vi "Configure Session.vi"(8 "error in":errorcluster, 11 "Plugin in":refnum<class "DateTimeChannel.lvclass">) -> (0 "error out":errorcluster, 3 "Plugin out":refnum<class "DateTimeChannel.lvclass">)   [LabVIEW 2023, in "DateTimeChannel.lvlib" / "DateTimeChannel.lvclass"]
uses:
  DateTimeChannel.lvclass
  C:/Program Files/National Instruments/LabVIEW 2023/vi.lib/FlexLogger/SDK/PluginSDK.lvlibp/PEFClasses/SDK/Plugin/Plugin.lvclass
  DateTimeChannel.lvclass/DateTimeChannel.ctl
  Date Time Channel Global.vi
  <vilib>/FlexLogger/SDK/PluginSDK.lvlibp/PEFClasses/SDK/Plugin/ParameterAccess/Read String.vi
  <vilib>/FlexLogger/SDK/PluginSDK.lvlibp/PEFClasses/SDK/Plugin/Plugin.lvclass
  C:/Program Files/National Instruments/LabVIEW 2023/vi.lib/FlexLogger/SDK/PluginSDK.lvlibp/PEFClasses/SDK/Processing Element/Processing Element.lvclass
  C:/dev/niflexlogger-plugins/plugins/DateTimeChannel/source/DateTimeChannel/DateTimeChannel.lvclass
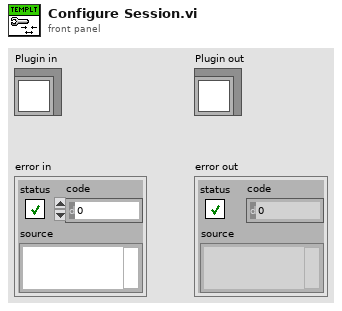
[diagram p1: front panel]
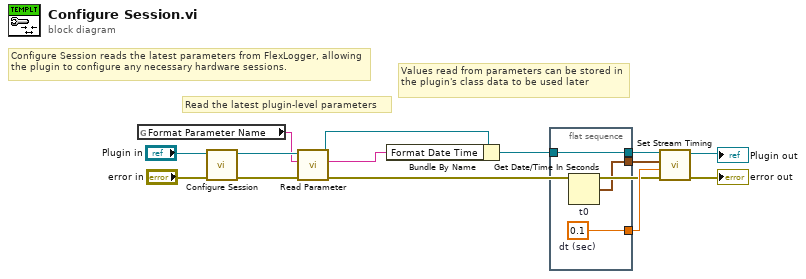
[diagram p0: block diagram]
diagram:
  # "Read the latest plugin-level parameters"
  # "Configure Session reads the latest parameters from FlexLogger, allowing the plugin to configure any necessary hardware sessions."
  # "Values read from parameters can be stored in the plugin's class data to be used later"
  n1 = global read "Date Time Channel Global.vi" "Format Parameter Name"() -> (w1:string)
  n2 = call-parent "Configure Session.vi"("error in (no error)"="error in", "Processing Element in"="Plugin in") -> ("error out"=w7:errorcluster, "Processing Element out"=w8:refnum<class "DateTimeChannel.lvclass">)  [unwired: 8 in]
  n3 = call-poly <vilib>:"Read Parameter.vi"("error in (no error)"=w7, "Name"=w1, "Plugin in"=w8) -> ("error out"=w4:errorcluster, "Value"=w5:string, "Plugin out"=w6:refnum<class "DateTimeChannel.lvclass">)  [unwired: 5 in, 1 out]
  n4 = Bundle By Name(cluster=w6, "Format Date Time"=w5) -> (w11:refnum<class "DateTimeChannel.lvclass">)
  n5 = flat-sequence {
    tunnel: [w17] -> w10
    tunnel: [w16] -> w9
    tunnel: w11 -> [w15]
    tunnel: [w15] -> w2
    frame #0 {
      w16 = 0.1  # dt (sec)
      n6 = Get Date/Time In Seconds "t0"() -> (seconds since 1Jan1904=w17:timestamp)
    }
  }
  n7 = call-dynamic "Set Stream Timing.vi"("error in (no error)"=w4, "dt(sec)"=w9, "Start Time"=w10, "Plugin in"=w2) -> ("error out"=→"error out":errorcluster, "Plugin out"=→"Plugin out":refnum<class "DateTimeChannel.lvclass">)  [unwired: 6 in]
